vi "Update test sequence step.vi"(5 "Disable \nprompt":bool, 9 "Result":bool=TRUE, 10 "Main Test Status":refnum<vi>, 11 "input cluster":T4={"User name"="", "user account"="", "UI"=[], "DI"=[], "Barcode"="", "MCListbox Ref_in"=refnum, "sequence step #"=0, "Result?"=FALSE, "Report Path"=path "", "Test Sequence"=enum."Ensure all the connections are OK", "skip Test  "=[FALSE, FALSE, FALSE, FALSE, FALSE, FALSE, FALSE, FALSE, FALSE, FALSE, FALSE, FALSE, FALSE, FALSE, FALSE, FALSE, FALSE, FALSE, FALSE, FALSE, FALSE, FALSE, FALSE, FALSE, FALSE, FALSE, FALSE, FALSE, FALSE, FALSE, FALSE, FALSE]} {"DI"."Upper limit" format="%#_7f"; "DI"."Lower limit" format="%#_7f"}) -> (2 "Main test sequence":T1, 3 "output cluster":T4={"User name"="", "user account"="", "UI"=[], "DI"=[], "Barcode"="", "MCListbox Ref_in"=refnum, "sequence step #"=0, "Result?"=FALSE, "Report Path"=path "", "Test Sequence"=enum."Ensure all the connections are OK", "skip Test  "=[FALSE, FALSE, FALSE, FALSE, FALSE, FALSE, FALSE, FALSE, FALSE, FALSE, FALSE, FALSE, FALSE, FALSE, FALSE, FALSE, FALSE, FALSE, FALSE, FALSE, FALSE, FALSE, FALSE, FALSE, FALSE, FALSE, FALSE, FALSE, FALSE, FALSE, FALSE, FALSE]} {"DI"."Upper limit" format="%#_7f"; "DI"."Lower limit" format="%#_7f"})   [LabVIEW 2021]
uses:
  5.ACTIVITIES/1.LabVIEW_State_Machine_Template/LabVIEW_State_Machine_Template/LabVIEW_State_Machine_Template/Project_Template/Queue Test updator/Controls/initialise cluster.ctl
  5.ACTIVITIES/1.LabVIEW_State_Machine_Template/LabVIEW_State_Machine_Template/LabVIEW_State_Machine_Template/Project_Template/Queue Test updator/Controls/test step description.ctl
  5.ACTIVITIES/1.LabVIEW_State_Machine_Template/LabVIEW_State_Machine_Template/LabVIEW_State_Machine_Template/Project_Template/Queue Test updator/Controls/comparison selection.ctl
  controls/Main test sequence.ctl
  <vilib>/Utility/miscctls.llb/LVRowAndColumnTypeDef.ctl
panel:
  out "error out":errorcluster
  out "DI 2":T2[](array[typedef]) {"Upper limit" format="%#_7f"; "Lower limit" format="%#_7f"}
  out "DI":T2[](array[typedef]) {"Upper limit" format="%#_7f"; "Lower limit" format="%#_7f"}
  out "Test Sequence 2":T1
  in  "Test Name":string
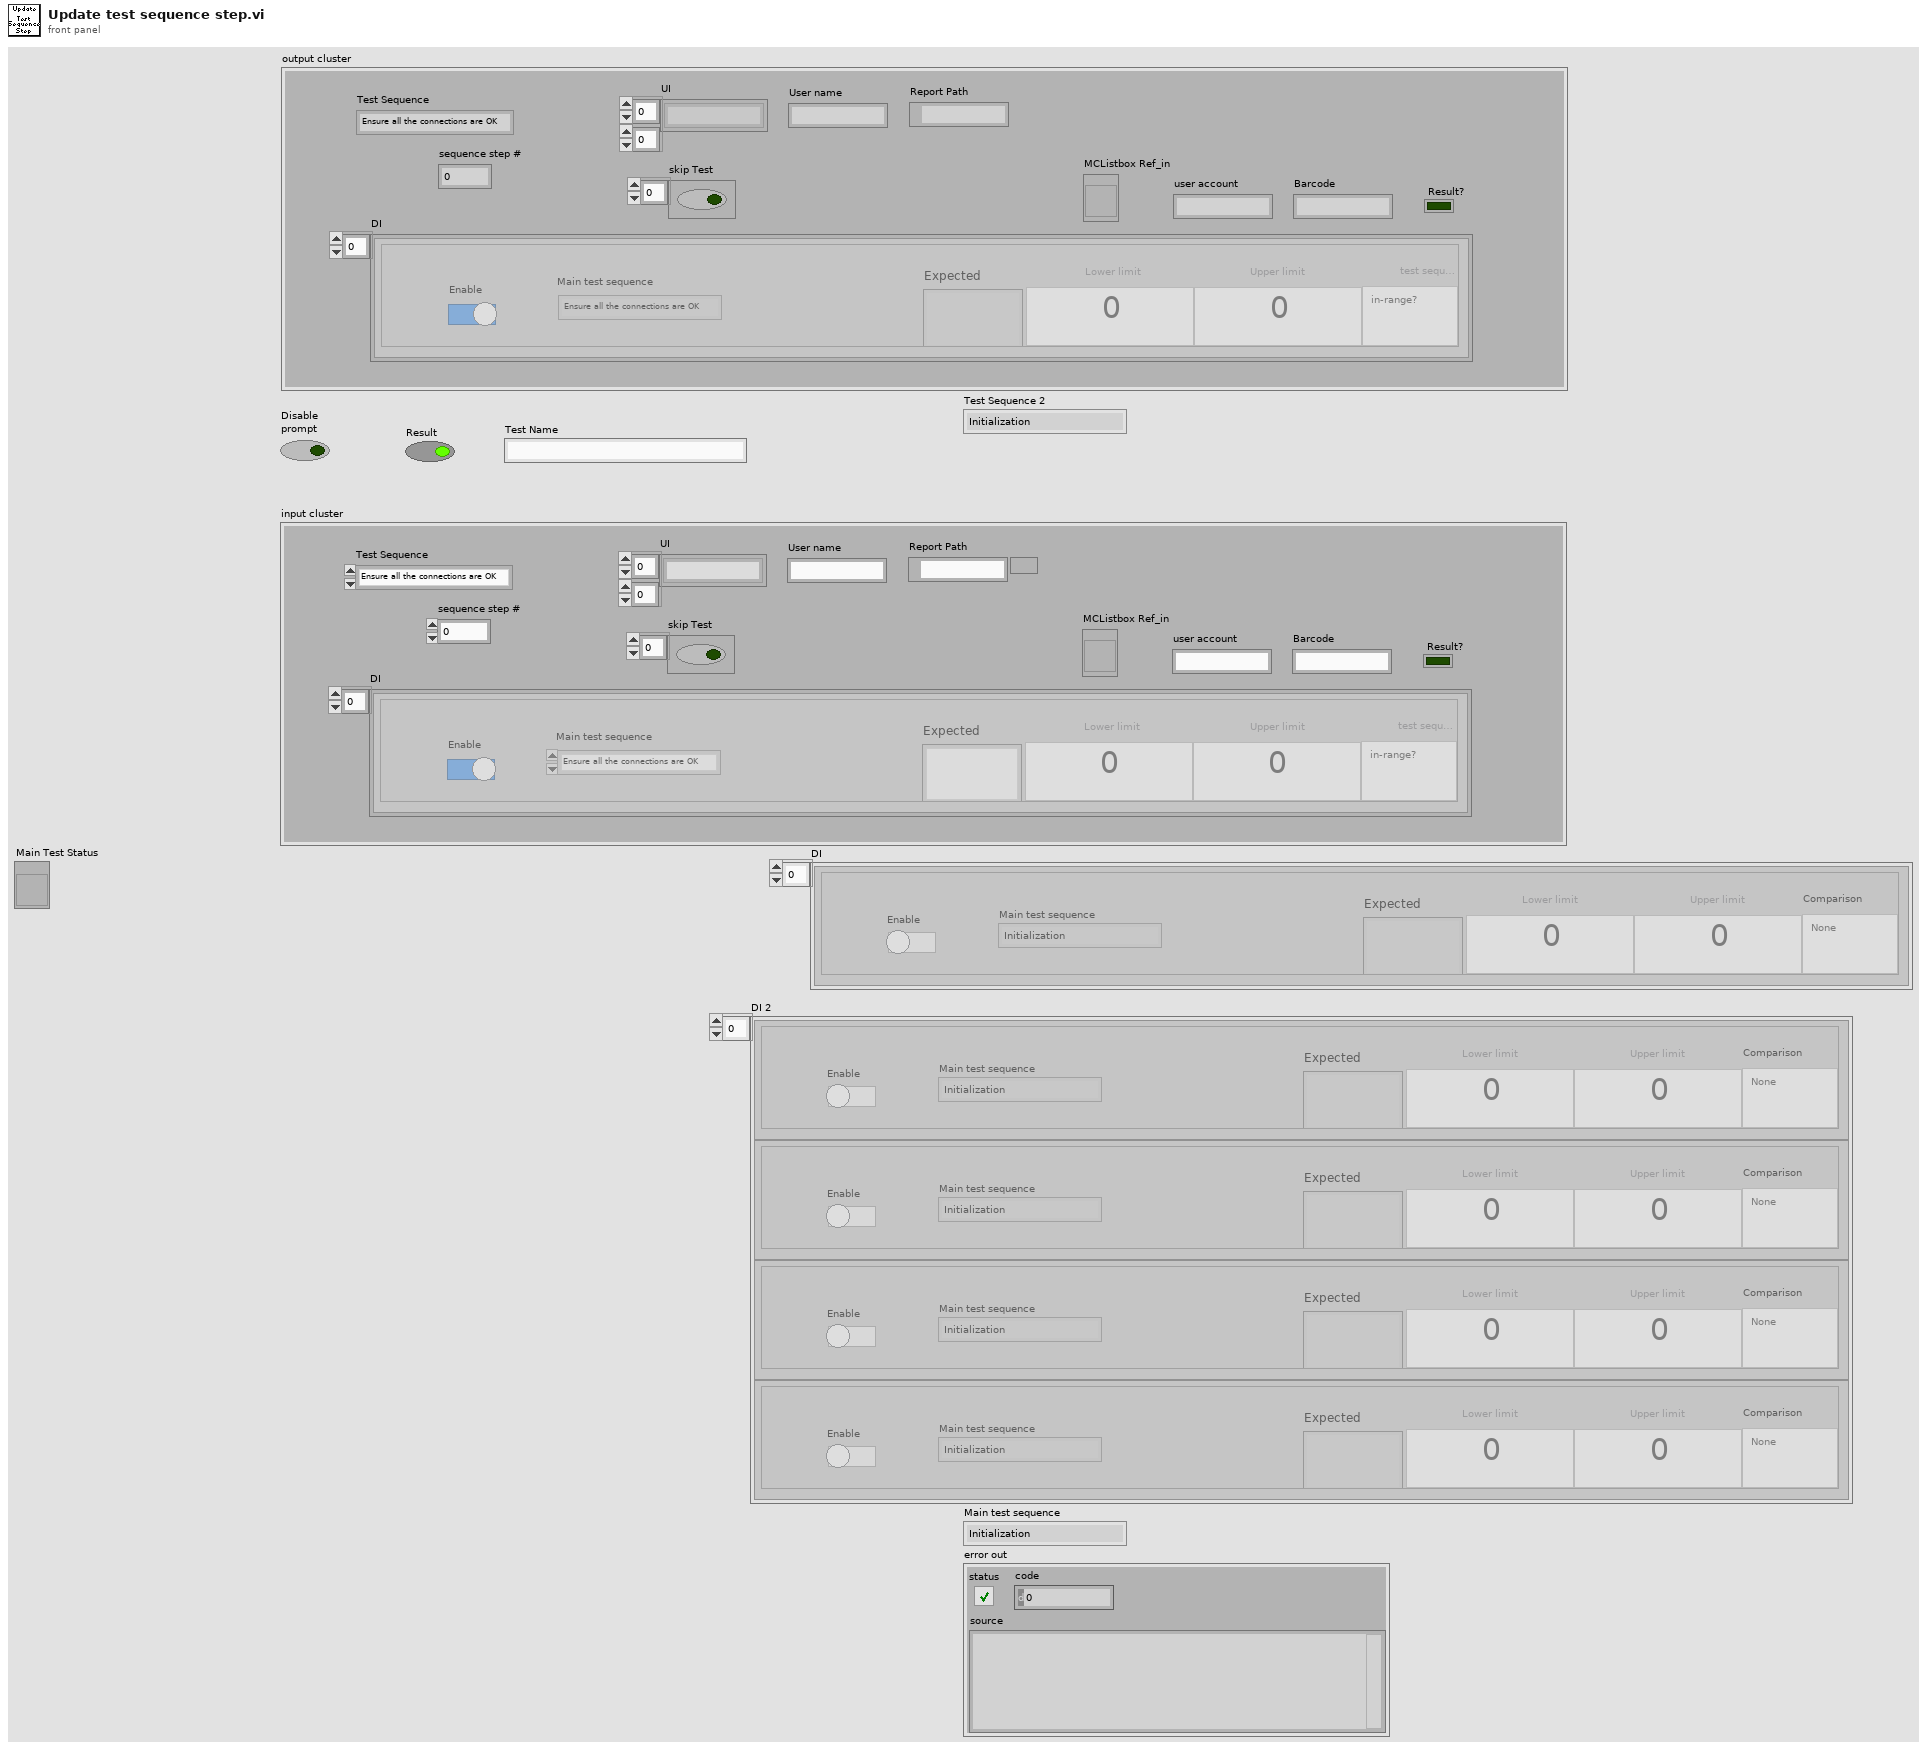
[diagram p1: front panel]
types:
  T1 = typedef "Main test sequence.ctl" = enum16{"Initialization", "Ensure all the connections are OK", "Turn ON 230V AC Input", "Load the Firmware", "Unlock_Opensesame & Stop console Logs", "Earth Detection", "Read Firmware", "Read & Write PCB Serial No", "Emergancy Switch Check", "Update WIFI credentials ", "Reboot", "Unlock Opensesame & Stop_console Logs", "WIFI State", "WIFI SSID", "Board revision", "ADC NTC Temp", "ADC_TYPE2_RCD_CURRENT", "5V Output Voltage", "3.3V Output Voltage", "D+M Sense", "Output Weld Sense", "FW Power Reset", "Unlock Opensesame & Stop console_Logs", "Reset switch Check", "Exit"}
  T2 = typedef "test step description.ctl" = cluster{"Lower limit":dbl, "Upper limit":dbl, "Comparison":T3, "Expected":string, "Enable":bool, "Main test sequence":T1}
  T3 = typedef "comparison selection.ctl" = enum16{"None", "in-range?", "less than?", "greater than?", "equal to?", "not equal to?", "less or equal to?", "greater or equal to?"}
  T4 = typedef "initialise cluster.ctl" = cluster{"User name":string, "user account":string, "UI":string[][], "DI":T2[], "Barcode":string, "MCListbox Ref_in":refnum<vi>, "sequence step #":u32, "Result?":bool, "Report Path":path, "Test Sequence":T1, "skip Test  ":bool[]}
  T5 = typedef "LVRowAndColumnTypeDef.ctl" = cluster{"Row":i32, "Column":i32}
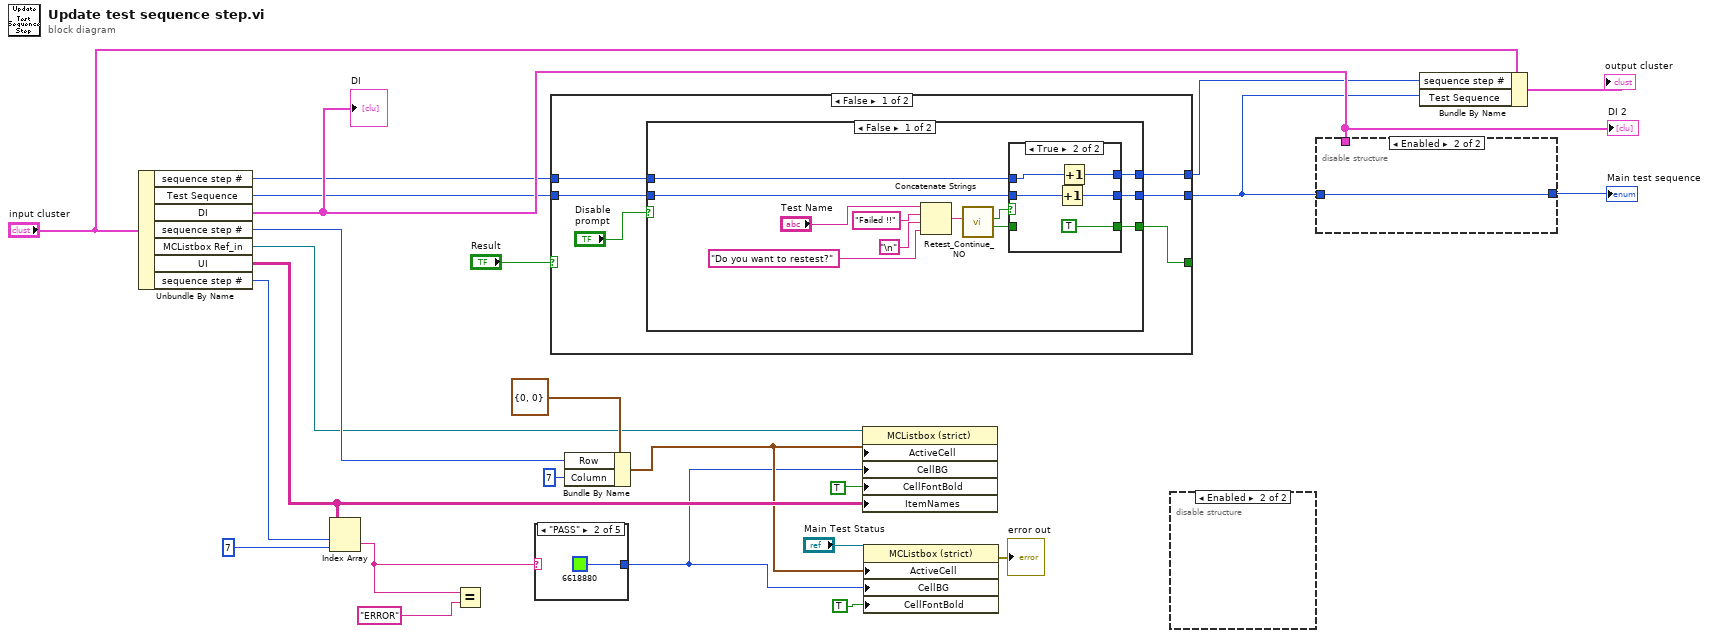
[diagram p0: block diagram]
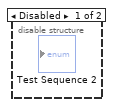
[diagram p2: hidden frame]
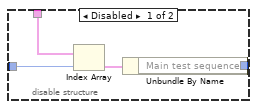
[diagram p3: hidden frame]
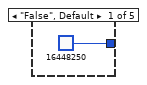
[diagram p4: hidden frame]
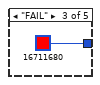
[diagram p5: hidden frame]
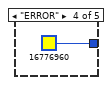
[diagram p6: hidden frame]
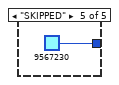
[diagram p7: hidden frame]
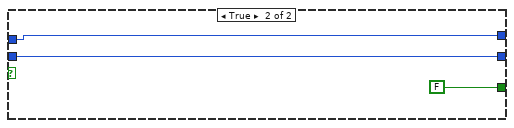
[diagram p9: hidden frame]
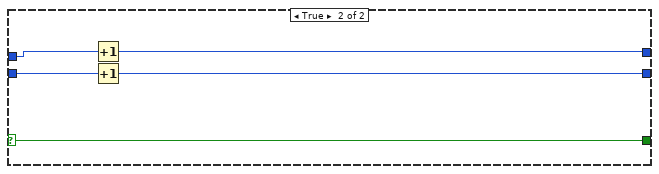
[diagram p10: hidden frame]
diagram:
  n1 = Unbundle By Name("input cluster") -> ("sequence step #"=w7:u32, "Test Sequence"=w9:T1, "DI"=w11:T2[], "sequence step #"=w22:u32, "MCListbox Ref_in"=w20:refnum<vi>, "UI"=w12:string[][], "sequence step #"=w15:u32)
  "DI" <- w11
  "DI 2" <- w11
  n2 = Index Array(array=w12, index (row)=w15, index (col)=7 ("Column")) -> (element=w17:string)
  n3 = Equal?(x=w17, y="ERROR") -> ()  [unwired: 1 out]
  n4 = case shown="\"PASS\"" w17 {
    tunnel: [u32 16448250 u32 6618880 u32 16711680 u32 16776960 u32 9567230] -> w4
    frame "False", Default {
    }
    frame "PASS" {
    }
    frame "FAIL" {
    }
    frame "ERROR" {
    }
    frame "SKIPPED" {
    }
  }
  n5 = case shown="False" "Result" {
    selector: "Result" -> [_ w61]
    tunnel: [w34 w63] -> w8
    tunnel: w9 -> [w33 w62]
    tunnel: [w35 w61] -> _
    tunnel: w7 -> [w31 w60]
    tunnel: [w30 w59] -> w6
    frame False {
      n6 = case shown="False" "Disable \nprompt" {
        tunnel: [w42 FALSE ("Boolean")] -> w35
        tunnel: [w40 w58] -> w34
        tunnel: w33 -> [w39 w58]
        tunnel: w31 -> [w37 w56]
        tunnel: [w36 w56] -> w30
        frame False {
          n7 = Concatenate Strings("Test Name", "Failed !!" ("string"), "\n", "Do you want to restest?" ("string")) -> (w43:string)
          n8 = call "Retest_Continue_NO.vi"("input string"=w43) -> ("Boolean"=w41:bool, "Continue 2"=w38:bool)  [unwired: 8 in, 1 out]
          n9 = case shown="True" w38 {
            tunnel: [w49 TRUE ("Boolean")] -> w42
            tunnel: w41 -> [w49 _]
            tunnel: [w50 w53] -> w40
            tunnel: w39 -> [w50 w54]
            tunnel: w37 -> [w48 w52]
            tunnel: [w48 w51] -> w36
            frame False {
            }
            frame True {
              n10 = Increment(x=w54) -> (x+1=w53:T1)
              n11 = Increment(x=w52) -> (x+1=w51:u32)
            }
          }
        }
        frame True {
        }
      }
    }
    frame True {
      n12 = Increment(x=w60) -> (x+1=w59:u32)
      n13 = Increment(x=w62) -> (x+1=w63:T1)
    }
  }
  n14 = Bundle By Name(cluster=T5 {"Row"=0, "Column"=0} ("Active Cell:Active Cell"), "Row"=w22, "Column"=7) -> (w5:T5)
  n15 = property class="MCListbox (strict)"(reference=w20, "ActiveCell"=w5, "CellBG"=w4, "CellFontBold"=TRUE ("Active Cell:Cell Font:Bold"), "ItemNames"=w12) -> ()  [unwired: 1 in, 2 out]
  n16 = property on="Property Node" class="MCListbox (strict)"(reference="Main Test Status", "ActiveCell"=w5, "CellBG"=w4, "CellFontBold"=TRUE ("Active Cell:Cell Font:Bold")) -> (error out=→"error out":errorcluster)  [unwired: 1 in, 1 out]
  n17 = disable-structure shown="Enabled" {
    frame Disabled {
    }
    frame Enabled {
    }
  }
  n18 = disable-structure shown="Enabled" {
    disable-tunnel: w8 -> [w67 w68]
    disable-tunnel: w11 -> [w66 _]
    disable-tunnel: [w65 w68] -> w10
    frame Disabled {
      n19 = Index Array(array=w66, index=w67) -> (element=w64:T2)
      n20 = Unbundle By Name(w64) -> ("Main test sequence"=w65:T1)
    }
    frame Enabled {
    }
  }
  "Main test sequence" <- w10
  n21 = Bundle By Name(cluster="input cluster", "sequence step #"=w6, "Test Sequence"=w8) -> (→"output cluster":T4)
